vi "mupSetVarValue.vi"(8 "error in (no error)":errorcluster, 10 "varValue":dbl, 11 "varAddr in":u64) -> (0 "error out":errorcluster, 3 "varAddr out":u64)   [LabVIEW 2018, in "mupLib.lvlib"]
doc: "Set the value of the variable at the specified memory location.\n\nUse the address returned by the <b>mupDefineVar</b> function as the input to <b>varAddr</b>."
uses:
  mupLib.lvlib
panel:
  # "Set the value of the variable at the specified memory location.\n\nUse the address returned by the mupDefineVar function as the input to varAddr."
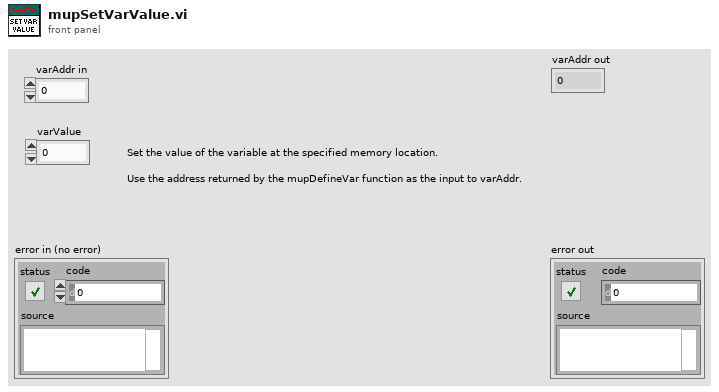
[diagram p1: front panel]
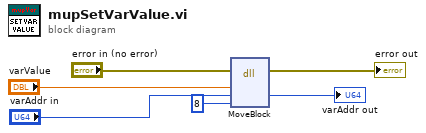
[diagram p0: block diagram]
diagram:
  n1 = dll-call lib="LabVIEW" fn="MoveBlock"(error in="error in (no error)", "ps"="varValue", "pd"="varAddr in", "size"=8) -> (error out=→"error out":errorcluster, "pd"=→"varAddr out":u64)  [unwired: 5 in, 1 out]
